vi "Update Log Path box colors.vi"(8 "error in (no error)":errorcluster, 9 "Force Default Colors? (F)":bool, 10 "Path Ref":refnum<vi>, 11 "Settings in":T1) -> (0 "error out":errorcluster, 3 "Settings out":T1)   [LabVIEW 2021, in "Settings.lvlib"]
doc: "Change the colors of the file path text box according to whether the data log file be overwritten: default colors when safe, red tint when overwriting."
uses:
  Settings.lvlib
  Settings.ctl
  Acquisition/Hardware Configuration.ctl
  Acquisition/Channel Settings.ctl
  Acquisition/IO Device.ctl
  Acquisition/Sensor Type.ctl
  Interval Timer/Repeat Interval.ctl
  Interval Timer/Interval Length.ctl
  Interval Timer/Interval Token.ctl
  Acquisition/IO API.ctl
  Logging/Logging Configuration.ctl
  Logging/Logging Mode.ctl
  Diagnostics/Diagnostics Configuration.ctl
  controls/Graph Settings.ctl
  <vilib>/Utility/miscctls.llb/LVTextColorsTypeDef.ctl
  Acquisition/Acquisition.lvlib
  Interval Timer/Interval Timer.lvlib
  Logging/Logging.lvlib
  Diagnostics/Diagnostics.lvlib
  Acquisition/IO Context.ctl
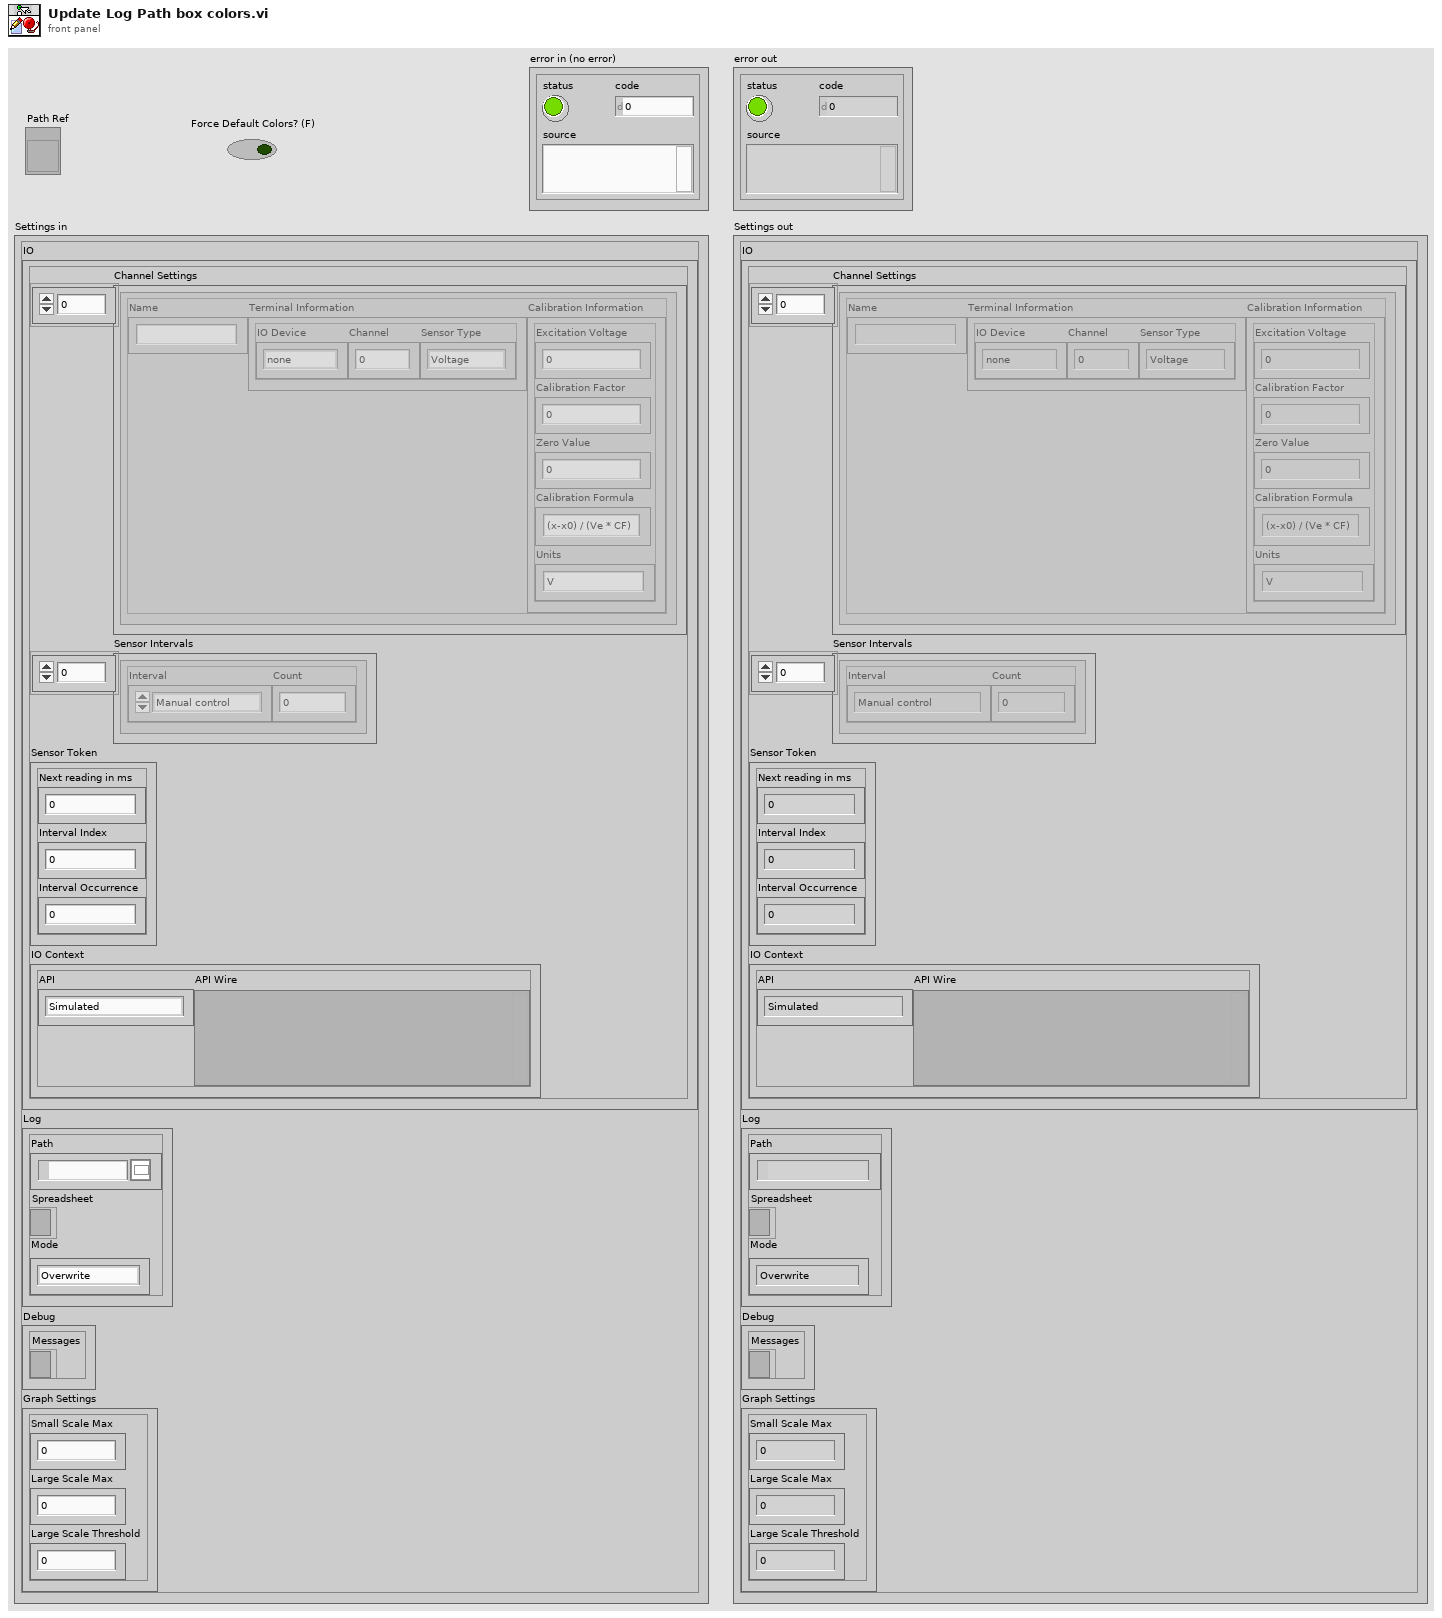
[diagram p1: front panel]
types:
  T1 = typedef "Settings.lvlib/Settings.ctl" = cluster{"IO":T2, "Log":T11, "Debug":T13, "Graph Settings":T14}
  T2 = typedef "Acquisition.lvlib/Hardware Configuration.ctl" = cluster{"Channel Settings":T3[], "Sensor Intervals":T6[], "Sensor Token":T8, "IO Context":T9}
  T3 = typedef "Acquisition.lvlib/Channel Settings.ctl" = cluster{"Name":string, "Terminal Information":cluster{"IO Device":T4, "Channel":i32, "Sensor Type":T5}, "Calibration Information":cluster{"Excitation Voltage":dbl, "Calibration Factor":dbl, "Zero Value":dbl, "Calibration Formula":string, "Units":string}}
  T4 = typedef "Acquisition.lvlib/IO Device.ctl" = enum16{"none", "9219", "9401"}
  T5 = typedef "Acquisition.lvlib/Sensor Type.ctl" = enum16{"Voltage", "Load", "Pressure", "Encoder"}
  T6 = typedef "Interval Timer.lvlib/Repeat Interval.ctl" = cluster{"Interval":T7, "Count":i32}
  T7 = typedef "Interval Timer.lvlib/Interval Length.ctl" = enum16{"Manual control", "1 second", "10 seconds", "30 seconds", "60 seconds", "600 seconds", "1200 seconds", "3600 seconds"}
  T8 = typedef "Interval Timer.lvlib/Interval Token.ctl" = cluster{"Next reading in ms":u32, "Interval Index":i32, "Interval Occurrence":i32}
  T9 = typedef "Acquisition.lvlib/IO Context.ctl" = cluster{"API":T10, "API Wire":variant}
  T10 = typedef "Acquisition.lvlib/IO API.ctl" = enum16{"Simulated", "DAQmx"}
  T11 = typedef "Logging.lvlib/Logging Configuration.ctl" = cluster{"Path":path, "Spreadsheet":refnum<file>, "Mode":T12}
  T12 = typedef "Logging.lvlib/Logging Mode.ctl" = enum16{"Overwrite", "Append", "Create New"}
  T13 = typedef "Diagnostics.lvlib/Diagnostics Configuration.ctl" = cluster{"Messages":refnum<file>}
  T14 = typedef "Graph Settings.ctl" = cluster{"Small Scale Max":dbl, "Large Scale Max":dbl, "Large Scale Threshold":dbl}
  T15 = typedef "LVTextColorsTypeDef.ctl" = cluster{"Text Color":u32, "Background Color":u32}
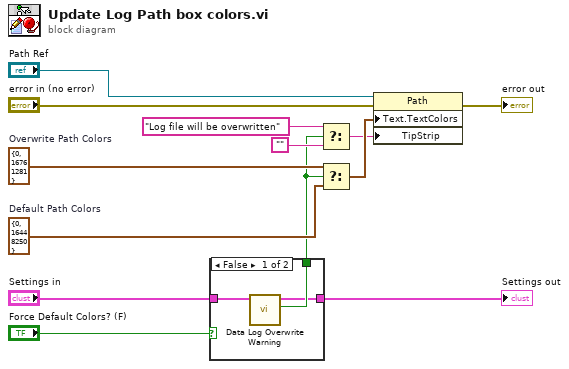
[diagram p0: block diagram]
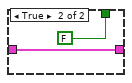
[diagram p2: hidden frame]
diagram:
  w11 = T15 {"Text Color"=0, "Background Color"=16448250}  # Default Path Colors
  w12 = T15 {"Text Color"=0, "Background Color"=16761281}  # Overwrite Path Colors
  n1 = case shown="False" "Force Default Colors? (F)" {
    tunnel: [w16 FALSE ("Overwrite Warning?")] -> w4
    tunnel: [w15 w18] -> w10
    tunnel: "Settings in" -> [w14 w18]
    frame False {
      n2 = call "Data Log Overwrite Warning.vi"("Settings in"=w14) -> ("Overwrite Warning?"=w16:bool, "Settings out"=w15:T1)  [unwired: 8 in, 1 out]
    }
    frame True {
    }
  }
  "Settings out" <- w10
  n3 = Select(t="Log file will be overwritten", s=w4, f="") -> (s? t:f=w5:string)
  n4 = Select(t=w12, s=w4, f=w11) -> (s? t:f=w13:T15)
  n5 = property on="Property Node" class="Path"(reference="Path Ref", error in="error in (no error)", "Text.TextColors"=w13, "TipStrip"=w5) -> (error out=→"error out":errorcluster)  [unwired: 1 out]
